vi "New.vi"(11 "triggers":refnum<class "RolloverTrigger.lvclass">[](array[class])) -> (3 "RolloverTrigger.Multi out":refnum<class "RolloverTrigger.Multi.lvclass">)   [LabVIEW 2018, in "GLog.lvlib" / "RolloverTrigger.Multi.lvclass"]
uses:
  RolloverTrigger.Multi.lvclass
  RolloverTrigger/RolloverTrigger.lvclass
  RolloverTrigger.Multi.lvclass/RolloverTrigger.Multi.ctl
panel:
  # "Connector Pane"
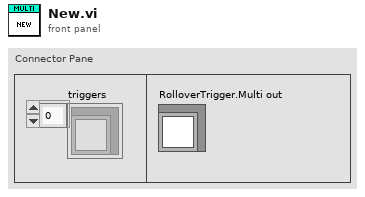
[diagram p1: front panel]
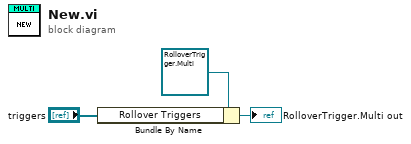
[diagram p0: block diagram]
diagram:
  n1 = Bundle By Name(cluster=refnum<class "RolloverTrigger.Multi.lvclass"> refnum ("RolloverTrigger.Multi in"), "Rollover Triggers"="triggers") -> (→"RolloverTrigger.Multi out":refnum<class "RolloverTrigger.Multi.lvclass">)
